vi "Run_after.vi"(8 "error in":errorcluster) -> (0 "error out":errorcluster)   [LabVIEW 2024]
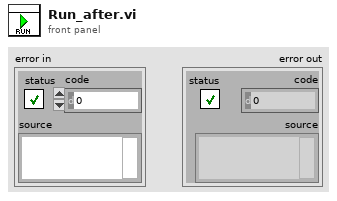
[diagram p1: front panel]
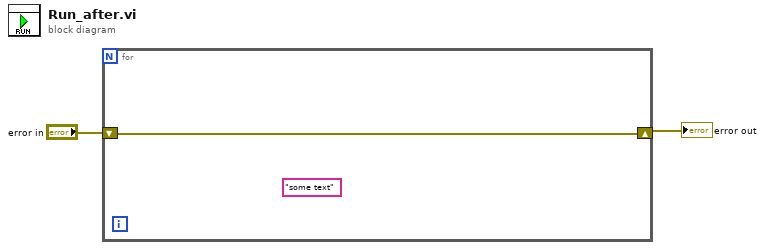
[diagram p0: block diagram]
diagram:
  n1 = for {
    shift-right: [w3] -> w1
    shift-left: "error in" -> [w3]
    (unwired) "some text"
  }
  "error out" <- w1
